vi "Good.vi"(0 "x":dbl) -> (4 "y":dbl)   [LabVIEW 2026, in "Lib.lvlib"]
doc: "Test fixture: calls Helper.vi."
uses:
  Lib.lvlib
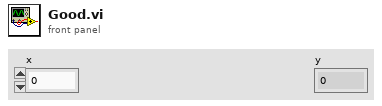
[diagram p1: front panel]
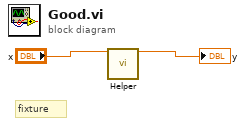
[diagram p0: block diagram]
diagram:
  # "fixture"
  n1 = call "Helper.vi"("x"="x") -> ("y"=→"y":dbl)  [unwired: 14 in]
